vi "SystemsUI.vi"() -> ()   [LabVIEW 2013, in "PL Framework Configuration Tool.lvlib" / "Systems.lvclass"]
doc: "This VI is a template of the minimun components for a node UI.\nIt shows how to use the queue and the user event."
uses:
  Systems.lvclass
  <vilib>/NI/Configuration Framework/Node/NodeRef.ctl
  <vilib>/NI/Configuration Framework/Node/NISE_CEF_Node.lvclass
  <vilib>/NI/AMC/Message Queue.ctl
  <vilib>/NI/AMC/Message.ctl
  <vilib>/NI/Tools/Keyed Array/KeyedArray.ctl
  <vilib>/NI/Configuration Framework/Node/UserEventRef.ctl
  <vilib>/NI/Configuration Framework/Controls/EventCluster.ctl
  <vilib>/NI/Configuration Framework/Node/RefreshUIEvent.ctl
  <vilib>/NI/Configuration Framework/Node/CacheState.ctl
  <vilib>/NI/Configuration Framework/Node/StopEvent.ctl
  <vilib>/NI/Configuration Framework/Node/NodeChangeEvent.ctl
  <vilib>/Utility/miscctls.llb/LVPositionTypeDef.ctl
  Systems.lvclass/Systems.ctl
  Framework Configuration Classes/system configuration/PL_System Configuration.lvclass/PL_System Configuration.ctl
  <vilib>/NI/Configuration Framework/serializable configuration/set alias.vi
  <vilib>/NI/Configuration Framework/serializable configuration/get alias.vi
  Framework Configuration Classes/system configuration/PL_System Configuration.lvclass
  <vilib>/NI/DCAF UI Toolkit/Controls/DCAF UI Elements.lvlib
  <vilib>/NI/Tools/Keyed Array/Tools_KeyedArray.lvlib
  <vilib>/NI/AMC/AMC.lvlib
  <vilib>/NI/Configuration Framework/NISE_CEF_TreeControl.lvlib
panel:
  in  "Top Level Tab Control":enum32{"Configuration Settings"}(tab)
  in  "Configuration Name":string
  in  "Major":u16=1 min=1
  in  "Minor":u16
  in  "Fix":u16
  in  "Build":u16=1 min=1
  in  "Description":string
  out "Time Last Saved 2":string
  in  "node change":T1
  in  "stop event":T2
  in  "cache state":T3
  in  "refresh UI":T4
  in  "user event":T5
  in  "main queue":T6
  in  "node ref":T7
  # "Revision"
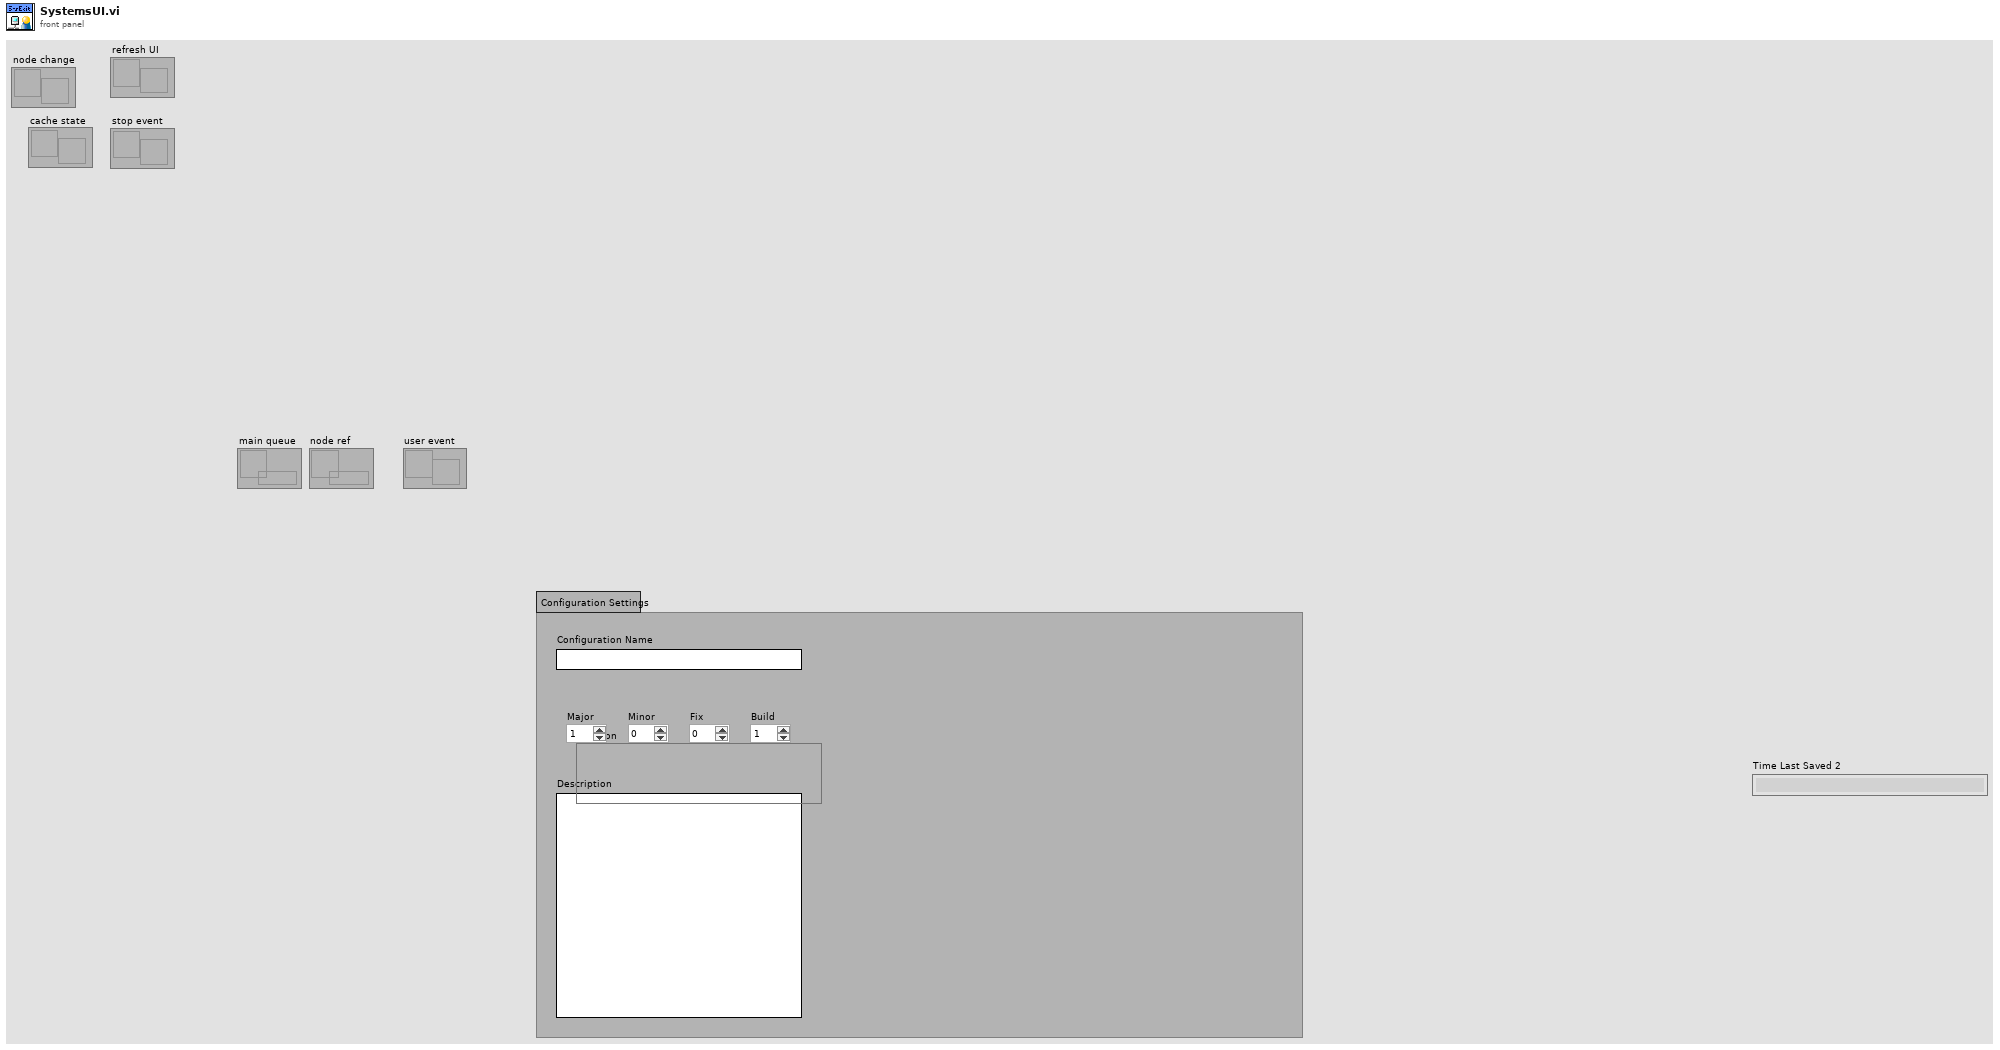
[diagram p1: front panel]
types:
  T1 = typedef "NISE_CEF_Node.lvclass/NodeChangeEvent.ctl" = refnum<user-event>
  T2 = typedef "NISE_CEF_Node.lvclass/StopEvent.ctl" = refnum<user-event>
  T3 = typedef "NISE_CEF_Node.lvclass/CacheState.ctl" = refnum<user-event>
  T4 = typedef "NISE_CEF_Node.lvclass/RefreshUIEvent.ctl" = refnum<user-event>
  T5 = typedef "NISE_CEF_Node.lvclass/UserEventRef.ctl" = refnum<user-event>
  T6 = typedef "AMC.lvlib/Message Queue.ctl" = refnum<queue>
  T7 = typedef "NISE_CEF_Node.lvclass/NodeRef.ctl" = refnum<data-value>
  T8 = typedef "LVPositionTypeDef.ctl" = cluster{"Left":i32, "Top":i32}
  T9 = cluster{"major":u16, "minor":u16, "fix":u16, "build":u16}
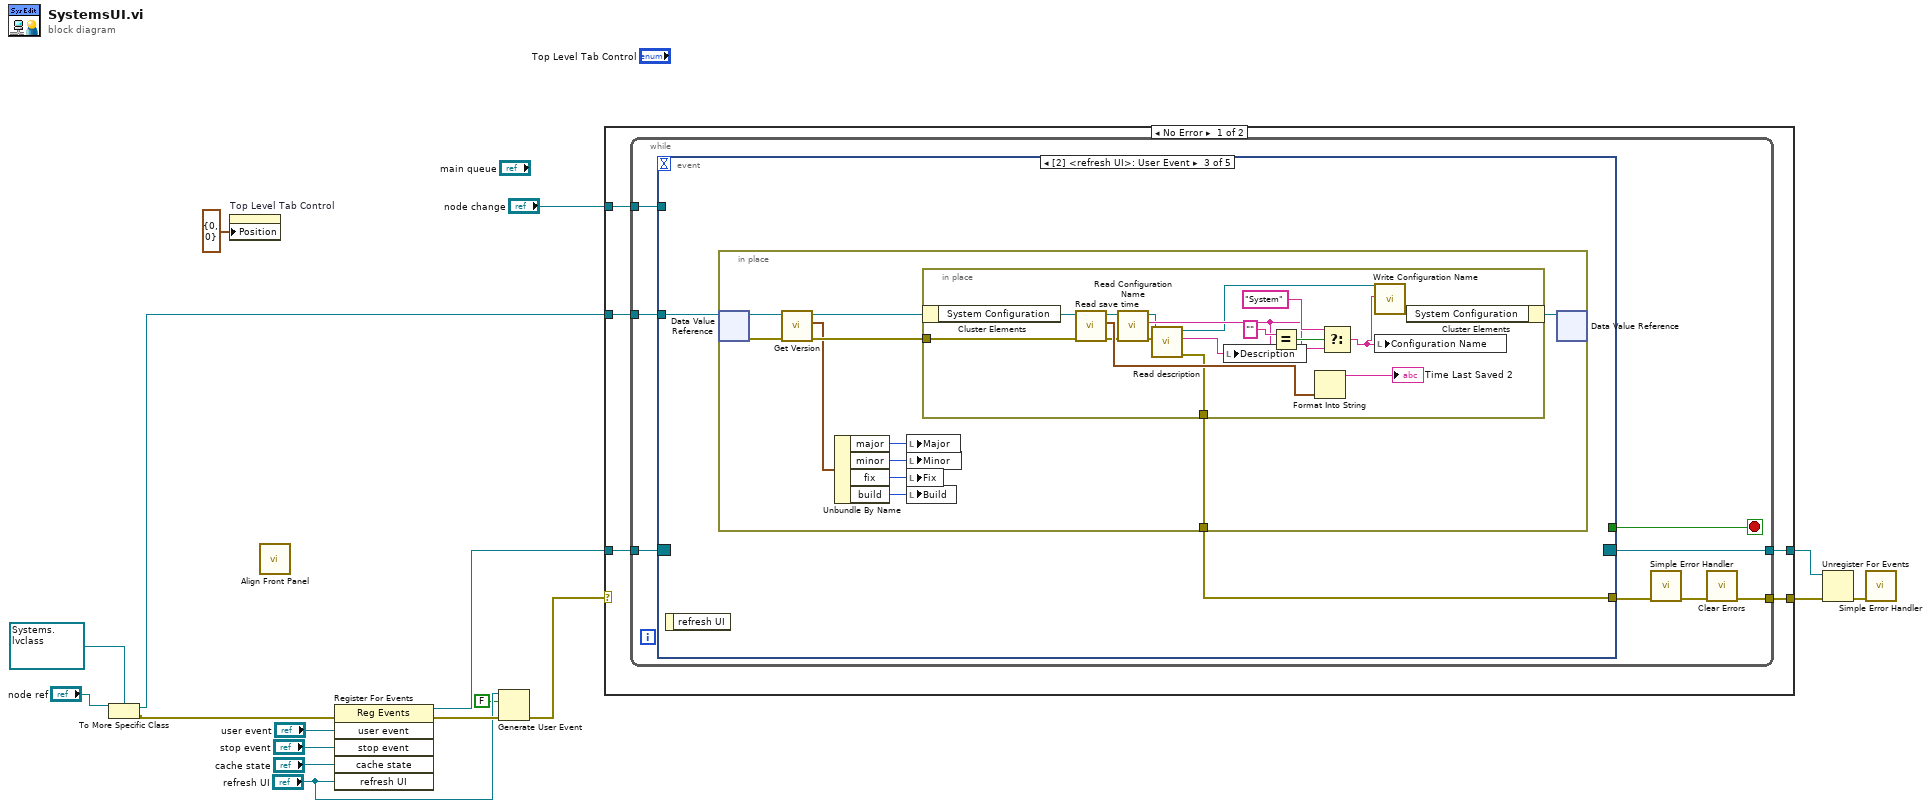
[diagram p0: block diagram]
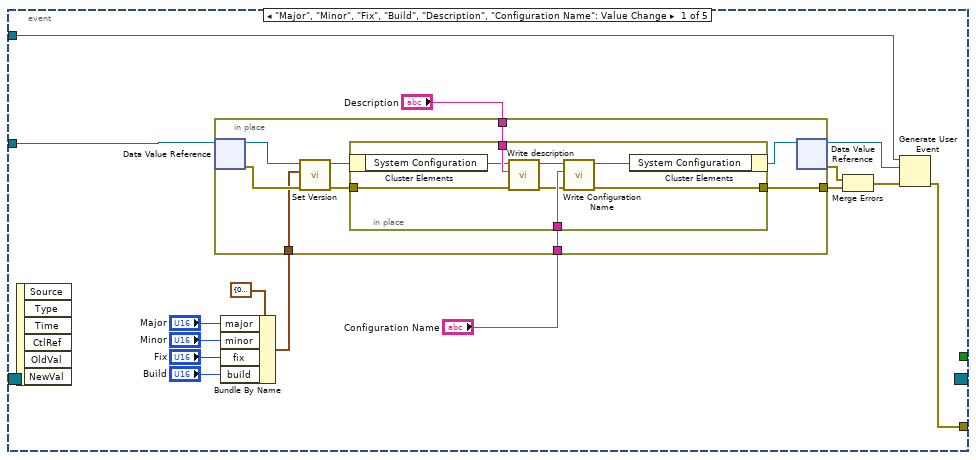
[diagram p2: hidden frame]
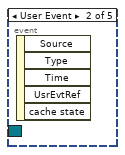
[diagram p3: hidden frame]
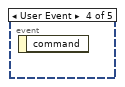
[diagram p4: hidden frame]
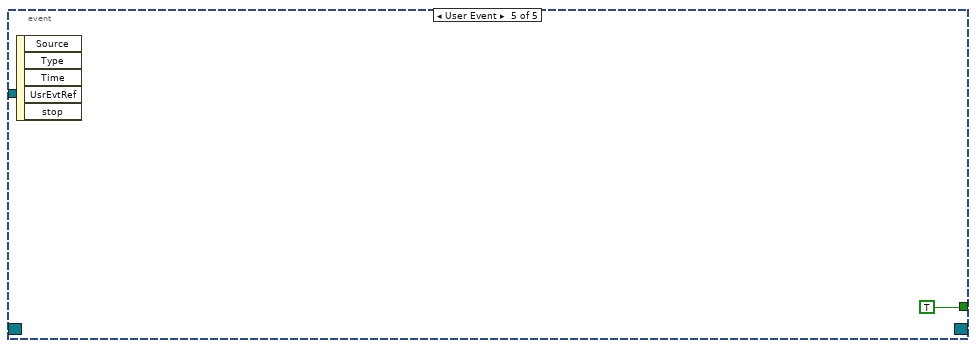
[diagram p5: hidden frame]
diagram:
  n1 = To More Specific Class(target class=refnum<data-value> refnum ("data value reference"), reference="node ref") -> (specific class reference=w2:refnum<data-value>, error out=w3:errorcluster)  [unwired: 1 in]
  n2 = property on="Top Level Tab Control" class="TabCtl (strict)"("Position"=T8 {"Left"=0, "Top"=0}) -> ()  [unwired: 2 in, 2 out]
  n3 = call <vilib>:"Align Front Panel.vi"() -> ()  [unwired: 10 in, 2 out]
  n4 = register-events(error in=w3, "user event", "stop event", "cache state", "refresh UI") -> (reference out=w16:refnum<event-registration>, error out=w13:errorcluster)  [unwired: 1 in]
  n5 = Generate User Event(user event="refresh UI", event data cluster=FALSE ("event data"), error in=w13) -> (error out=w5:errorcluster)  [unwired: 1 in, 1 out]
  n6 = case shown="No Error" w5 {
    selector: w5 -> [_ w95]
    tunnel: w2 -> [w22 _]
    tunnel: w16 -> [w21 w94]
    tunnel: [w20 w94] -> w15
    tunnel: [w19 w95] -> w14
    tunnel: "node change" -> [w18 _]
    frame No Error {
      n7 = while {
        tunnel: w22 -> [w30]
        tunnel: w21 -> [w29]
        tunnel: [w28] -> w20
        tunnel: [w23] -> w19
        tunnel: w18 -> [w25]
        stop <- w27 stop-if-true
        n8 = event shown="[2] <refresh UI>: User Event" {
          selector: w29 -> [_ _ _ _ _]
          dyn-events: [_ _ _ _ _] -> w28
          timeout: _ -> [_ _ _ _ _]
          tunnel: w30 -> [w45 _ w63 _ _]
          tunnel: [_ _ _ _ TRUE] -> w27
          tunnel: [w37 _ w64 _ _] -> w26
          tunnel: w25 -> [w39 _ _ _ _]
          event "Major", "Minor", "Fix", "Build", "Description", "Configuration Name": Value Change {
            n9 = event-data() -> ()  [unwired: 1 in, 6 out]
            n10 = Bundle By Name(cluster=T9 {"major"=0, "minor"=0, "fix"=0, "build"=0} ("version"), "major"="Major", "minor"="Minor", "fix"="Fix", "build"="Build") -> (w31:T9)
            n11 = in-place {
              in-place-border: "Description" -> [w53]
              in-place-border: "Configuration Name" -> [w52]
              in-place-border: [w51] -> w42
              in-place-border: w31 -> [w46]
              n12 = in-place-dvr #1(w45) -> (w47:refnum<class "Systems.lvclass">, w48:errorcluster)
              n13 = call "Set Version.vi"("error in (no error)"=w48, "version"=w46, "system in"=w47) -> ("error out"=w50:errorcluster, "system out"=w49:refnum<class "Systems.lvclass">)  [unwired: 7 in]
              n14 = in-place {
                in-place-border: w53 -> [w62]
                in-place-border: w52 -> [w59]
                in-place-border: w50 -> [w55]
                in-place-border: [w57] -> w51
                n15 = in-place-cluster #2(w49) -> ("System Configuration"=w56:refnum<class "PL_System Configuration.lvclass">)
                n16 = call "Write description.vi"("error in"=w55, "description"=w62, "PL_System Configuration in"=w56) -> ("error out"=w58:errorcluster, "PL_System Configuration out"=w61:refnum<class "PL_System Configuration.lvclass">)  [unwired: 7 in]
                n17 = call "Write Configuration Name.vi"("error in"=w58, "Configuration Name"=w59, "PL_System Configuration in"=w61) -> ("error out"=w57:errorcluster, "PL_System Configuration out"=w60:refnum<class "PL_System Configuration.lvclass">)  [unwired: 7 in]
                n18 = in-place-cluster #2("System Configuration"=w60) -> (w54:refnum<class "Systems.lvclass">)
              }
              n19 = in-place-dvr #1(w54) -> (w38:refnum<data-value>, w41:errorcluster)
            }
            n20 = Merge Errors(w41, w42) -> (w40:errorcluster)
            n21 = Generate User Event(user event=w39, event data cluster=w38, error in=w40) -> (error out=w37:errorcluster)  [unwired: 1 in, 1 out]
          }
          event User Event {
            n22 = event-data() -> ()  [unwired: 1 in, 5 out]
          }
          event User Event {
            n23 = event-data() -> ()  [unwired: 1 in, 1 out]
            n24 = in-place {
              in-place-border: [w74] -> w64
              n25 = in-place-dvr #3(w63) -> (w73:refnum<class "Systems.lvclass">, w72:errorcluster)
              n26 = call "Get Version.vi"("error in (no error)"=w72, "system in"=w73) -> ("error out"=w70:errorcluster, "version"=w69:T9, "system out"=w71:refnum<class "Systems.lvclass">)  [unwired: 7 in]
              n27 = Unbundle By Name(w69) -> ("major"=w65:u16, "minor"=w66:u16, "fix"=w67:u16, "build"=w68:u16)
              n28 = local write "Major"(w65) -> ()
              n29 = local write "Minor"(w66) -> ()
              n30 = local write "Fix"(w67) -> ()
              n31 = local write "Build"(w68) -> ()
              n32 = in-place {
                in-place-border: w70 -> [w78]
                in-place-border: [w76] -> w74
                n33 = in-place-cluster #4(w71) -> ("System Configuration"=w77:refnum<class "PL_System Configuration.lvclass">)
                n34 = call "Read save time.vi"("error in"=w78, "PL_System Configuration in"=w77) -> ("error out"=w84:errorcluster, "save time"=w87:timestamp, "PL_System Configuration out"=w85:refnum<class "PL_System Configuration.lvclass">)  [unwired: 7 in]
                n35 = call "Read Configuration Name.vi"("error in"=w84, "PL_System Configuration in"=w85) -> ("error out"=w86:errorcluster, "Configuration Name"=w88:string, "PL_System Configuration out"=w83:refnum<class "PL_System Configuration.lvclass">)  [unwired: 7 in]
                n36 = call "Read description.vi"("error in"=w86, "PL_System Configuration in"=w83) -> ("error out"=w76:errorcluster, "description"=w81:string, "PL_System Configuration out"=w82:refnum<class "PL_System Configuration.lvclass">)  [unwired: 7 in]
                n37 = local write "Description"(w81) -> ()
                n38 = Equal?(x="" ("y"), y=w88) -> (x = y?=w92:bool)
                n39 = Format Into String(w87) -> (resulting string=→"Time Last Saved 2":string)  [unwired: 3 in, 1 out]
                n40 = Select(t="System", s=w92, f=w88) -> (s? t:f=w79:string)
                n41 = call "Write Configuration Name.vi"("Configuration Name"=w79, "PL_System Configuration in"=w82) -> ("PL_System Configuration out"=w80:refnum<class "PL_System Configuration.lvclass">)  [unwired: 8 in, 1 out]
                n42 = local write "Configuration Name"(w79) -> ()
                n43 = in-place-cluster #4("System Configuration"=w80) -> (w75:refnum<class "Systems.lvclass">)
              }
              n44 = in-place-dvr #3(w75) -> ()  [unwired: 2 out]
            }
          }
          event User Event {
            n45 = event-data() -> ()  [unwired: 1 in, 1 out]
          }
          event User Event {
            n46 = event-data() -> ()  [unwired: 1 in, 5 out]
          }
        }
        n47 = call <vilib>:"Simple Error Handler.vi"("error in (no error)"=w26) -> ("error out"=w24:errorcluster)  [unwired: 4 in, 4 out]
        n48 = call <vilib>:"Clear Errors.vi"("error in (no error)"=w24) -> ("error out"=w23:errorcluster)  [unwired: 6 in]
      }
    }
    frame Error {
    }
  }
  n49 = Unregister For Events(event registration refnum=w15, error in=w14) -> (error out=w4:errorcluster)
  n50 = call <vilib>:"Simple Error Handler.vi"("error in (no error)"=w4) -> ()  [unwired: 4 in, 5 out]
